vi "Init.vi"(8 "error in (no error)":errorcluster, 9 "Config File Path":path=path "", 10 "Name":string, 11 "Process In":refnum<class "Process.lvclass">) -> (0 "error out":errorcluster, 3 "Process Out":refnum<class "Process.lvclass">)   [LabVIEW 2020, in "Process.lvclass"]
doc: "Initializes the process and creates necessary references. Anything initialized here is released in the Clear.vi method."
uses:
  Process.lvclass
  Process.lvclass/Process.ctl
  Protected/Messaging/Message Cluster.ctl
  Public/Lifecycle/Lifecycle State.ctl
  Base/Base.lvclass
  <vilib>/ErrorRing/Error Ring.xnode
  Protected/Broadcasting/Broadcast Message Cluster.ctl
  <vilib>/Utility/error.llb/Error Cluster From Error Code.vi
  Callback/Callback.lvclass
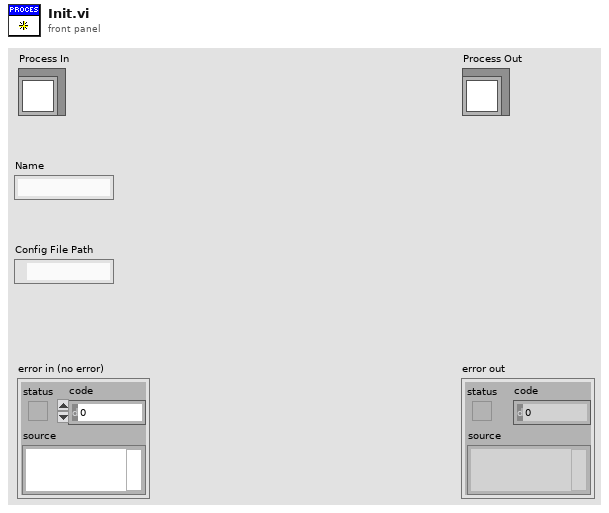
[diagram p1: front panel]
types:
  T1 = typedef "Process.lvclass/Lifecycle State.ctl" = enum16{"Uninitialized", "Initialized", "Started", "Running", "Stopped", "Finished"}
  T2 = typedef "Process.lvclass/Broadcast Message Cluster.ctl" = cluster{"Sender":string, "Message":string, "Message Data":variant}
  T3 = typedef "Process.lvclass/Message Cluster.ctl" = cluster{"Message":string, "Message Data":variant, "Request Callback":refnum<class "Callback.lvclass">}
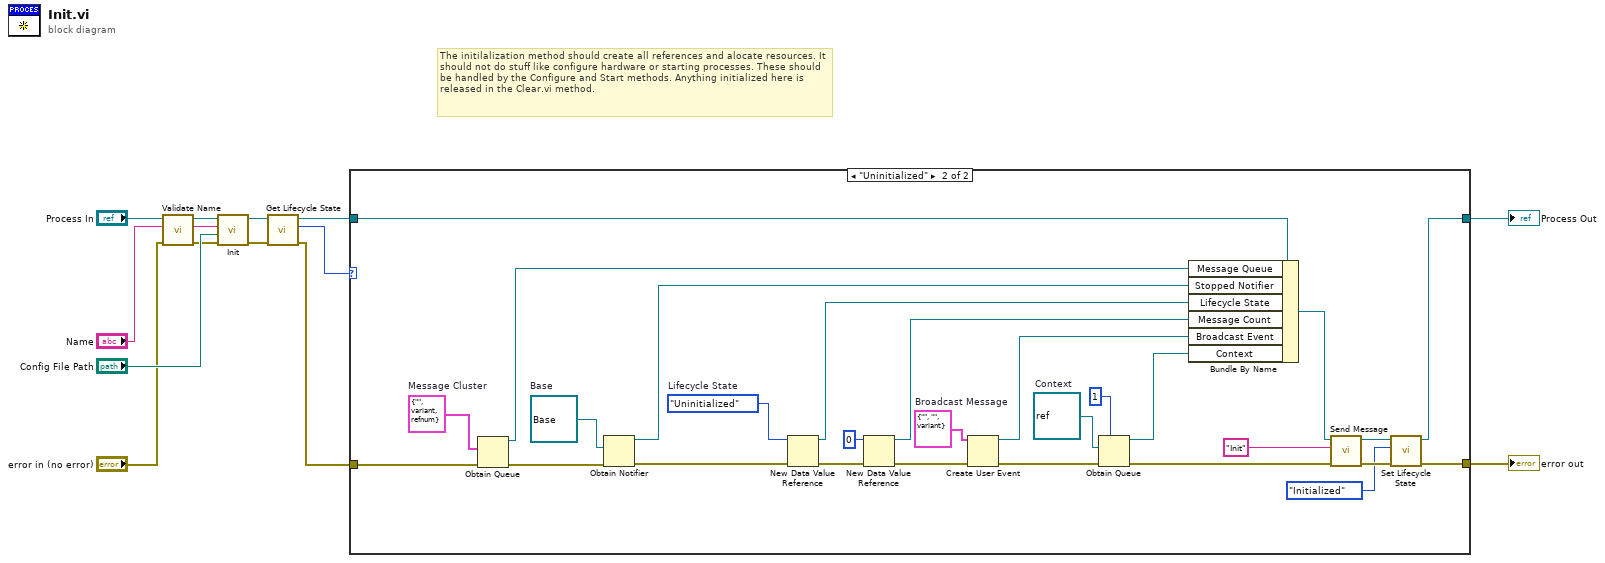
[diagram p0: block diagram]
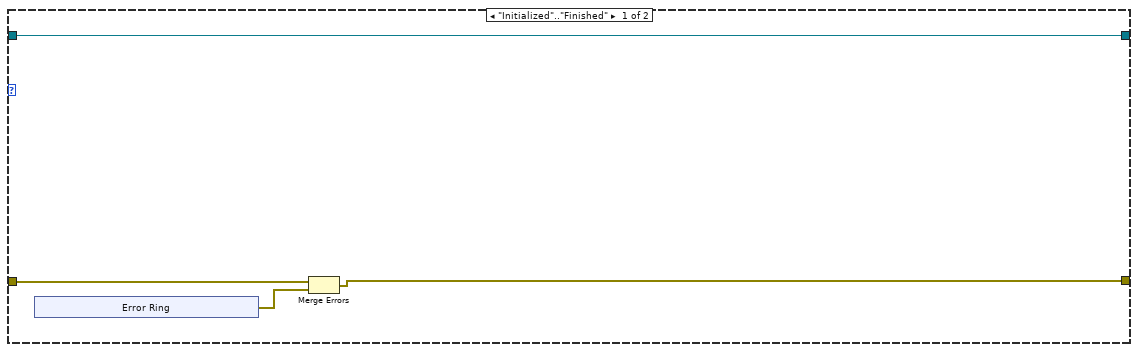
[diagram p2: hidden frame]
diagram:
  # "The initilalization method should create all references and alocate resources. It should not do stuff like configure hardware or starting processes. These should be handled by the Configure and Start methods. Anything initialized here is released in the Clear.vi method."
  n1 = call "Validate Name.vi"("error in (no error)"="error in (no error)", "Name In"="Name", "Process In"="Process In") -> ("error out"=w2:errorcluster, "Name Out"=w3:string, "Process Out"=w5:refnum<class "Process.lvclass">)  [unwired: 6 in]
  n2 = call-parent "Init.vi"("error in (no error)"=w2, "Config File Path"="Config File Path", "Name"=w3, "Base In"=w5) -> ("error out"=w8:errorcluster, "Base Out"=w10:refnum<class "Process.lvclass">)  [unwired: 6 in]
  n3 = call "Get Lifecycle State.vi"("error in (no error)"=w8, "Process In"=w10) -> ("error out"=w7:errorcluster, "Lifecycle State"=w13:T1, "Process Out"=w14:refnum<class "Process.lvclass">)  [unwired: 6 in, 1 out]
  n4 = case shown="\"Uninitialized\"" w13 {
    tunnel: [w18 w44] -> w12
    tunnel: [w15 w41] -> w11
    tunnel: w14 -> [w18 w35]
    tunnel: w7 -> [w16 w34]
    frame "Initialized".."Finished" {
      n5 = xnode "Error Ring"() -> ("error out"=w17:errorcluster)
      n6 = Merge Errors(w16, w17) -> (w15:errorcluster)
    }
    frame "Uninitialized" {
      w29 = refnum<class> refnum  # Context
      w33 = T2 {"Sender"="", "Message"="", "Message Data"=variant}  # Broadcast Message
      w37 = refnum<class "Base.lvclass"> refnum  # Base
      w46 = Lifecycle_State."Uninitialized"  # Lifecycle State
      w40 = T3 {"Message"="", "Message Data"=variant, "Request Callback"=refnum}  # Message Cluster
      n7 = Obtain Queue(element data type=w40, error in (no error)=w34) -> (queue out=w50:refnum<queue>, error out=w39:errorcluster)  [unwired: 3 in, 1 out]
      n8 = Obtain Notifier(notification data type=w37, error in (no error)=w39) -> (notifier out=w36:refnum<notifier>, error out=w47:errorcluster)  [unwired: 2 in, 1 out]
      n9 = New Data Value Reference(data value=w46, error in=w47) -> (data value reference=w45:refnum<data-value>, error out=w25:errorcluster)
      n10 = New Data Value Reference(data value=0, error in=w25) -> (data value reference=w23:refnum<data-value>, error out=w24:errorcluster)
      n11 = Create User Event(user event datatype=w33, error in=w24) -> (user event=w32:refnum<user-event>, error out=w31:errorcluster)
      n12 = Obtain Queue(max queue size (-1, unlimited)=1, element data type=w29, error in (no error)=w31) -> (queue out=w27:refnum<queue>, error out=w30:errorcluster)  [unwired: 2 in, 1 out]
      n13 = Bundle By Name(cluster=w35, "Message Queue"=w50, "Stopped Notifier"=w36, "Lifecycle State"=w45, "Message Count"=w23, "Broadcast Event"=w32, "Context"=w27) -> (w38:refnum<class "Process.lvclass">)
      n14 = call "Send Message.vi"("error in (no error)"=w30, "Message"="Init", "Process In"=w38) -> ("error out"=w43:errorcluster, "Process Out"=w49:refnum<class "Process.lvclass">)  [unwired: 7 in]
      n15 = call "Set Lifecycle State.vi"("error in (no error)"=w43, "Lifecycle State"=Lifecycle_State."Initialized", "Process In"=w49) -> ("error out"=w41:errorcluster, "Process Out"=w44:refnum<class "Process.lvclass">)  [unwired: 7 in]
    }
  }
  "error out" <- w11
  "Process Out" <- w12
